vi "HostMem Create_Size.vi"(6 "cvType":T1, 8 "error in (no error)":errorcluster, 9 "Rows":i32, 10 "Cols":i32, 11 "AllocType":T2) -> (0 "error out":errorcluster, 3 "HostMem":refnum<class "HostMem.lvclass">)   [LabVIEW 2020, in "OpenLvVision_OpenCv.lvlib" / "Cuda.lvlib" / "HostMem.lvclass"]
doc: "Object by Reference!\nCreates from host memory with the given size."
uses:
  HostMem.lvclass
  C:/Users/lukas/Documents/OpenLvVision_OpenCv/SourceCode/LabView/OpenLvVision_OpenCv/_LvHelpers/EdvrObject/EdvrObject.lvclass
  TypeDef/cvType.ctl
  _LvHelpers/EdvrObject/TypeDef/Edvr.ctl
  _LvHelpers/EdvrObject/EdvrObject.lvclass/EdvrObject.ctl
  _LvHelpers/EdvrObject/EdvrObject.lvclass
  OpenLvVision_OpenCv.lvlib
  <vilib>/ErrorRing/Error Ring.xnode
  <vilib>/Utility/error.llb/Error Cluster From Error Code.vi
  Dlls/OlvOpenCvWrapper.dll
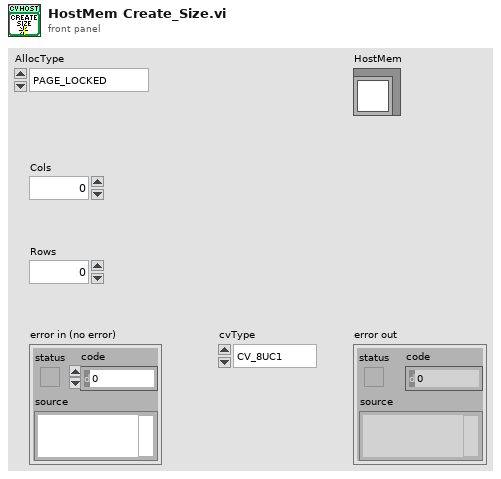
[diagram p1: front panel]
types:
  T1 = typedef "OpenLvVision_OpenCv.lvlib/cvType.ctl" = enum32{"CV_8UC1", "CV_8SC1", "CV_16UC1", "CV_16SC1", "CV_32SC1", "CV_32FC1", "CV_64FC1", "CV_16FC1", "CV_8UC2", "CV_8SC2", "CV_16UC2", "CV_16SC2", "CV_32SC2", "CV_32FC2", "CV_64FC2", "CV_16FC2", "CV_8UC3", "CV_8SC3", "CV_16UC3", "CV_16SC3", "CV_32SC3", "CV_32FC3", "CV_64FC3", "CV_16FC3", "CV_8UC4", "CV_8SC4", "CV_16UC4", "CV_16SC4", "CV_32SC4", "CV_32FC4", "CV_64FC4", "CV_16FC4"}
  T2 = typedef "OpenLvVision_OpenCv.lvlib/AllocType" = enum16{"PAGE_LOCKED", "SHARED", "WRITE_COMBINED"}
  T3 = typedef "OpenLvVision_OpenCv.lvlib/EdvrObject.lvclass/Edvr.ctl" = refnum<data-value>
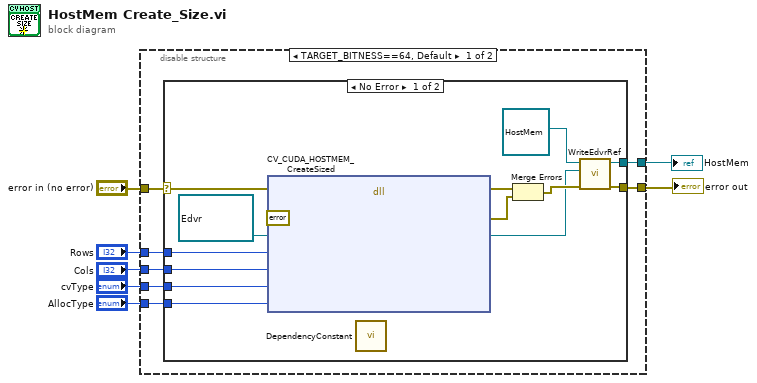
[diagram p0: block diagram]
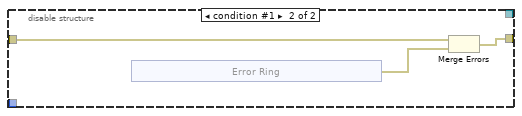
[diagram p3: hidden frame]
diagram:
  n1 = disable-structure shown="TARGET_BITNESS==64, Default" {
    disable-tunnel: "error in (no error)" -> [w14 w31]
    disable-tunnel: [w13 _] -> w6
    disable-tunnel: [w12 w32] -> w5
    disable-tunnel: "AllocType" -> [w11 _]
    disable-tunnel: "Cols" -> [w10 _]
    disable-tunnel: "Rows" -> [w9 _]
    disable-tunnel: "cvType" -> [w8 _]
    frame condition #0 (active) {
      n2 = case shown="No Error" w14 {
        selector: w14 -> [w21 w29]
        tunnel: [w28 w29] -> w12
        tunnel: [w27 _] -> w13
        tunnel: w11 -> [w18 _]
        tunnel: w10 -> [w17 _]
        tunnel: w9 -> [w16 _]
        tunnel: w8 -> [w15 _]
        frame No Error {
          n3 = dll-call lib="C:/Users/lukas/Documents/OpenLvVision_OpenCv/SourceCode/LabView/OpenLvVision_OpenCv/Dlls/OlvOpenCvWrapper.dll" fn="CV_CUDA_HOSTMEM_CreateSized"(error in=w21, "Error"=errorcluster {"status"=FALSE, "code"=0, "source"=""} ("error out"), "edvrRef"=T3 refnum ("Edvr"), "rows"=w16, "cols"=w17, "cvType"=w15, "allocType"=w18) -> (error out=w25:errorcluster, "Error"=w24:errorcluster, "edvrRef"=w20:T3)  [unwired: 7 in, 1 out]
          n4 = call "DependencyConstant.vi"() -> ()  [unwired: 12 in]
          n5 = Merge Errors(w25, w24) -> (w22:errorcluster)
          n6 = call "WriteEdvrRef.vi"("error in (no error)"=w22, "Edvr"=w20, "EdvrObject in"=refnum<class "HostMem.lvclass"> refnum ("OpenLvVision_OpenCv.lvlib:HostMem")) -> ("error out"=w28:errorcluster, "EdvrObject out"=w27:refnum<class "HostMem.lvclass">)  [unwired: 7 in]
        }
        frame Error {
        }
      }
    }
    frame condition #1 {
      n7 = xnode "Error Ring"() -> ("error out"=w30:errorcluster)
      n8 = Merge Errors(w31, w30) -> (w32:errorcluster)
    }
  }
  "error out" <- w5
  "HostMem" <- w6
